vi "VTU_Sensitivity_Calc.vi"(8 "error in (no error)":errorcluster={"status"=FALSE, "code"=0, "source"="\"\""}, 10 "acceptance formula":string, 11 "Initial/final lever and hitch values":string) -> (0 "error out":errorcluster={"status"=FALSE, "code"=0, "source"="\"\""}, 2 "status ok":bool, 3 "Sensitivity metrics and status":string)   [LabVIEW 2026]
doc: "INTENT: Optional VTU calculation plugin. LOGIC: Compute delta lever, delta hitch and configured sensitivity ratio/difference with unit checks."
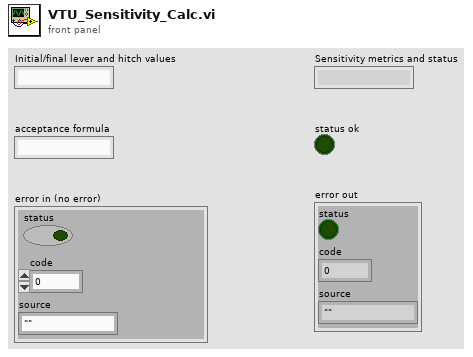
[diagram p1: front panel]
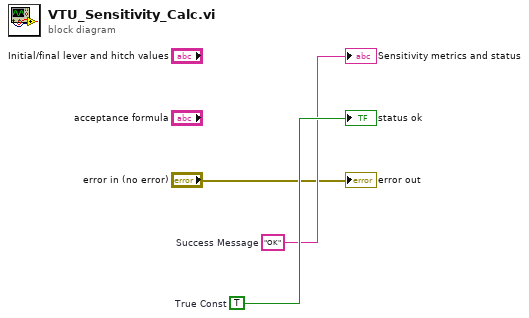
[diagram p0: block diagram]
diagram:
  w3 = TRUE  # True Const
  w2 = "OK"  # Success Message
  "Sensitivity metrics and status" <- w2
  "status ok" <- w3
  "error out" <- "error in (no error)"
